vi "Progress Fixture Record.vi"(8 "error in":errorcluster, 10 "set?":bool, 11 "record in":string) -> (0 "error out":errorcluster, 3 "record out":string)   [LabVIEW 2020, in "MCP Server tests.lvlib"]
doc: "Test helper (functional global). fake tool progress.vi stores here what it did: {\"steps\":n,\"cancelled\":true|false}, n being the number of steps it finished before it stopped. set? TRUE stores record in; FALSE reads. Tests reset it with set? TRUE and an empty record."
uses:
  MCP Server tests.lvlib
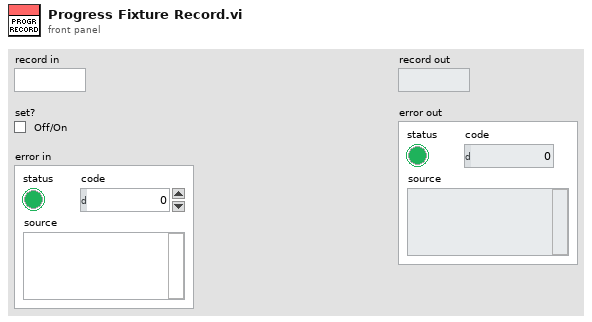
[diagram p1: front panel]
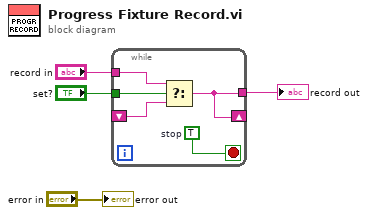
[diagram p0: block diagram]
diagram:
  n1 = while {
    tunnel: "record in" -> [w9]
    tunnel: "set?" -> [w8]
    shift-right: [w5] -> _
    shift-left: _ -> [w7]
    tunnel: [w5] -> w2
    stop <- w6 stop-if-true
    w6 = TRUE  # stop
    n2 = Select(t=w9, s=w8, f=w7) -> (s? t:f=w5:string)
  }
  "record out" <- w2
  "error out" <- "error in"
